vi "RemoteVI Windows Message.vi"(0 "windows":T1(array[cluster])) -> (4 "message":string)   [LabVIEW 2020, in "RemoteVI.lvlib"]
doc: "Builds the text message windows <json> (docs\\protocol.md section 7) from the window list of RemoteVI List Windows.vi: a JSON array, front-most window first, one object per window with id, title, x, y, w, h, modal, active and closable in that order - windows [] when there is none. title is taken as it is, already a JSON string literal (RemoteVI JSON String.vi), so the message is ASCII. The JSON is written field by field rather than with Flatten To JSON: the title has to stay the escaped literal it is (Flatten To JSON would escape its backslashes again), and the field order and spelling are the protocol's. Pure function, cannot fail. Reference: windowsMessage() in tools\\lib\\protocol.mjs."
uses:
  RemoteVI.lvlib
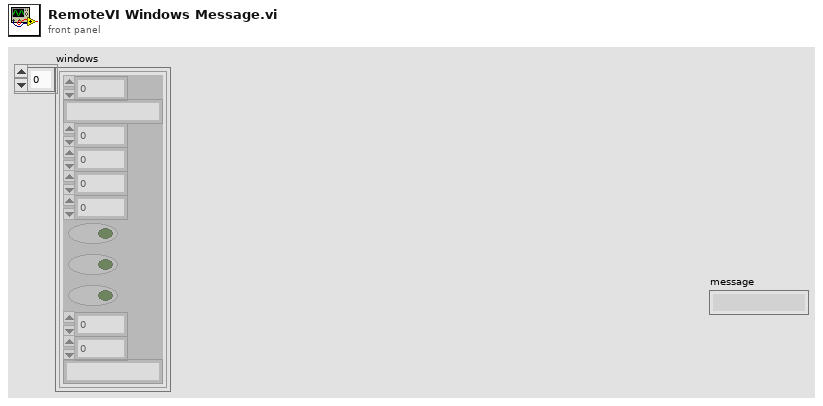
[diagram p1: front panel]
types:
  T1 = cluster{"id":u64, "title":string, "x":i32, "y":i32, "w":i32, "h":i32, "modal":bool, "active":bool, "closable":bool, "sx":i32, "sy":i32, "class":string}[]
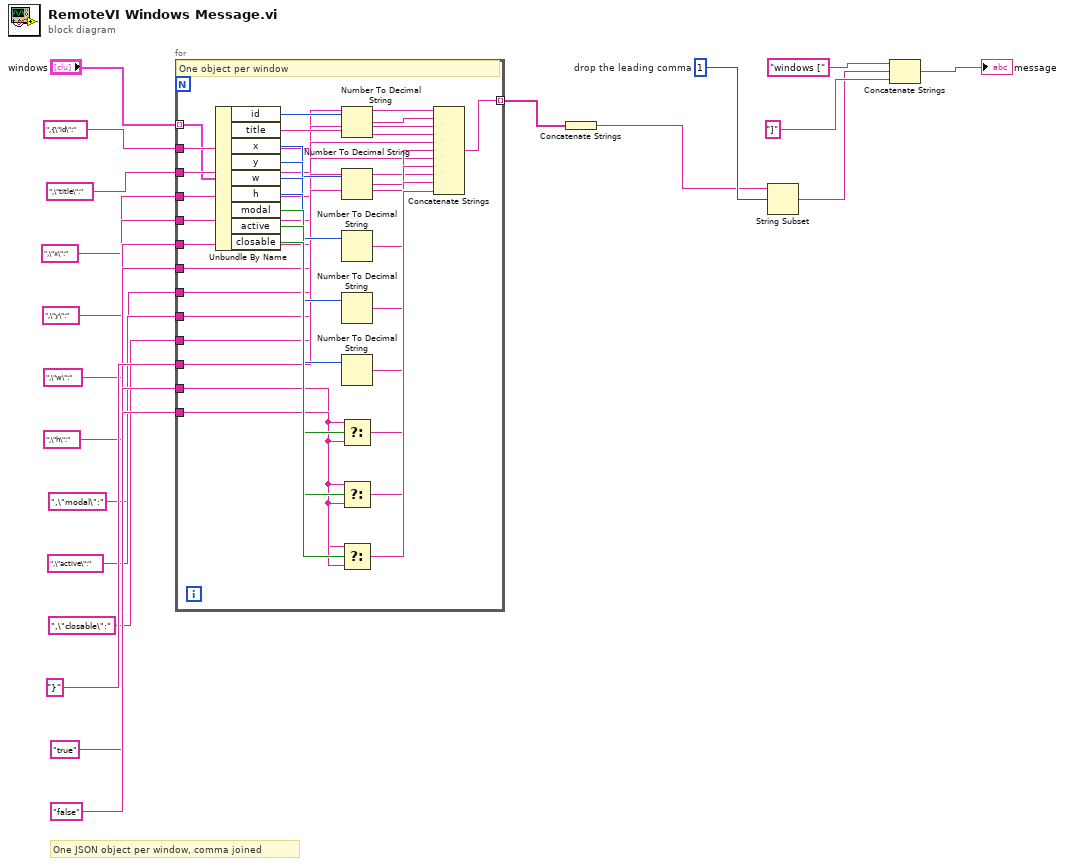
[diagram p0: block diagram]
diagram:
  w16 = 1  # drop the leading comma
  # "One JSON object per window, comma joined"
  n1 = for {
    tunnel: "windows" -> [w21] mode=indexing
    tunnel: ",{\"id\":" -> [w22]
    tunnel: ",\"title\":" -> [w23]
    tunnel: ",\"x\":" -> [w24]
    tunnel: ",\"y\":" -> [w25]
    tunnel: ",\"w\":" -> [w26]
    tunnel: ",\"h\":" -> [w27]
    tunnel: ",\"modal\":" -> [w28]
    tunnel: ",\"active\":" -> [w29]
    tunnel: ",\"closable\":" -> [w30]
    tunnel: "}" -> [w31]
    tunnel: "true" -> [w32]
    tunnel: "false" -> [w33]
    tunnel: [w51] -> w14 mode=indexing
    # "One object per window"
    n2 = Unbundle By Name(w21) -> ("id"=w34:u64, "title"=w35:string, "x"=w36:i32, "y"=w37:i32, "w"=w38:i32, "h"=w39:i32, "modal"=w40:bool, "active"=w41:bool, "closable"=w42:bool)
    n3 = Number To Decimal String(number=w34) -> (decimal integer string=w43:string)  [unwired: 1 in]
    n4 = Number To Decimal String(number=w36) -> (decimal integer string=w44:string)  [unwired: 1 in]
    n5 = Number To Decimal String(number=w37) -> (decimal integer string=w45:string)  [unwired: 1 in]
    n6 = Number To Decimal String(number=w38) -> (decimal integer string=w46:string)  [unwired: 1 in]
    n7 = Number To Decimal String(number=w39) -> (decimal integer string=w47:string)  [unwired: 1 in]
    n8 = Select(t=w32, s=w40, f=w33) -> (s? t:f=w48:string)
    n9 = Select(t=w32, s=w41, f=w33) -> (s? t:f=w49:string)
    n10 = Select(t=w32, s=w42, f=w33) -> (s? t:f=w50:string)
    n11 = Concatenate Strings(w22, w43, w23, w35, w24, w44, w25, w45, w26, w46, w27, w47, w28, w48, w29, w49, w30, w50, w31) -> (w51:string)
  }
  n12 = Concatenate Strings(w14) -> (w15:string)
  n13 = String Subset(string=w15, offset (0)=w16) -> (substring=w17:string)  [unwired: 1 in]
  n14 = Concatenate Strings("windows [", w17, "]") -> (→"message":string)
